vi "Eval_MultiVar_BulkMode.vi"(8 "error in (no error)":errorcluster, 9 "varValues":dbl[][](array[numeric]) format="%#_13g", 10 "varNames":string[](array[string]), 11 "muExpr in":refnum<class "mupExpr.lvclass">) -> (0 "error out":errorcluster, 2 "Result":dbl[](array[numeric]) format="%#_13g", 3 "muExpr out":refnum<class "mupExpr.lvclass">)   [LabVIEW 2015, in "mupExpr.lvclass"]
doc: "Update the value of multiple variables then evaluate the expression in bulk mode. Returns the array of results.\n\nNote that the array of values provided for variable values should be of size:\nNum Rows: Number of Variables\nNum Cols: Bulk Size\n\nIf any variable is not found, a warning is generated.\n\nIf multiple expressions have been input, the result of the last one in the list is returned."
uses:
  mupExpr.lvclass
  mupExpr.lvclass/mupExpr.ctl
  mupLib/mupSetVarValue_Array.vi
  mupLib/mupCheckError.vi
  <vilib>/Utility/error.llb/Error Cluster From Error Code.vi
  mupLib/mupLib.lvlib
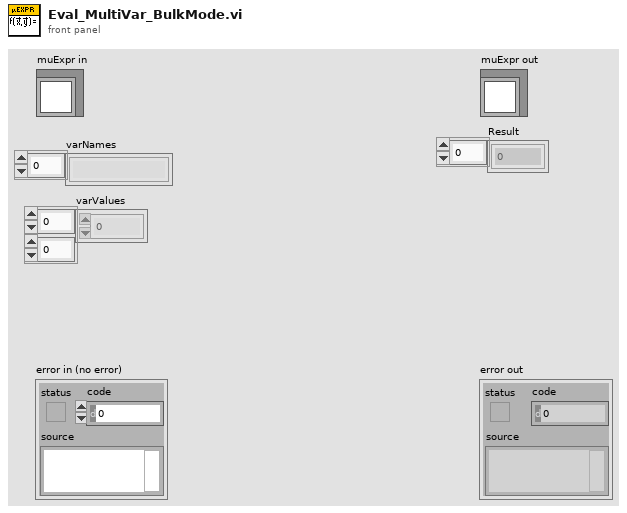
[diagram p1: front panel]
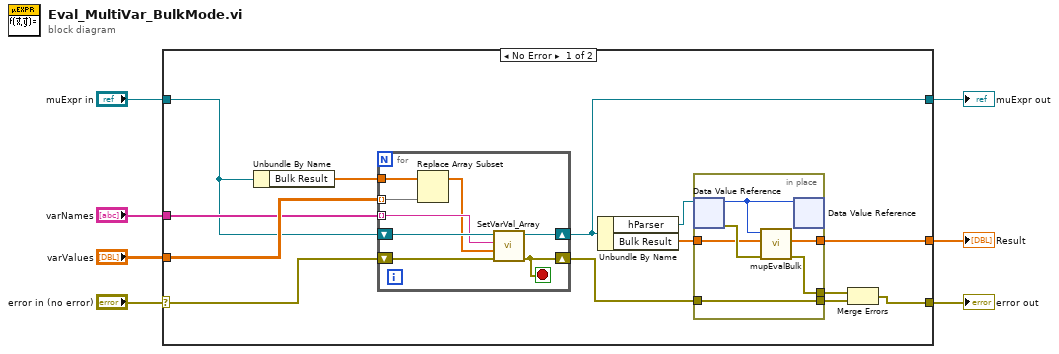
[diagram p0: block diagram]
diagram:
  n1 = case shown="No Error" "error in (no error)" {
    selector: "error in (no error)" -> [w17 w36]
    tunnel: "varValues" -> [w19 _]
    tunnel: "varNames" -> [w18 _]
    tunnel: [w12 _] -> w6
    tunnel: "muExpr in" -> [w16 w35]
    tunnel: [w9 w36] -> w4
    tunnel: [w13 w35] -> w3
    frame No Error {
      n2 = Unbundle By Name(w16) -> ("Bulk Result"=w20:dbl[])
      n3 = for {
        tunnel: w18 -> [w31] mode=indexing
        tunnel: w19 -> [w30] mode=indexing
        shift-right: [w27] -> w14
        shift-left: w17 -> [w33]
        tunnel: w20 -> [w34]
        shift-right: [w28] -> w13
        shift-left: w16 -> [w32]
        stop <- w27 stop-if-true
        n4 = Replace Array Subset(array=w34, new element=w30) -> (w29:dbl[])  [unwired: 1 in]
        n5 = call "SetVarVal_Array.vi"("error in (no error)"=w33, "varValue"=w29, "varName"=w31, "muExpr in"=w32) -> ("error out"=w27:errorcluster, "muExpr out"=w28:refnum<class "mupExpr.lvclass">)  [unwired: 6 in]
      }
      n6 = Unbundle By Name(w13) -> ("hParser"=w15:refnum<data-value>, "Bulk Result"=w8:dbl[])
      n7 = in-place {
        in-place-border: w14 -> [w22]
        in-place-border: [w26] -> w12
        in-place-border: [w23] -> w11
        in-place-border: [w22] -> w10
        in-place-border: w8 -> [w21]
        n8 = in-place-dvr #1(w15) -> (w24:u64, w25:errorcluster)
        n9 = call "mupEvalBulk.vi"("error in (no error)"=w25, "a_res"=w21, "hParser in"=w24) -> ("error out"=w23:errorcluster, "results"=w26:dbl[])  [unwired: 6 in, 1 out]
        n10 = in-place-dvr #1(w24) -> ()  [unwired: 2 out]
      }
      n11 = Merge Errors(w11, w10) -> (w9:errorcluster)
    }
    frame Error {
    }
  }
  "error out" <- w4
  "muExpr out" <- w3
  "Result" <- w6
